vi "Delete Unicode Header.vi"(1 "String in":string) -> (0 "String out":string)   [LabVIEW 2019, in "Language Editor.lvlib"]
doc: "- - -\nCopyright (c) 2026, Merecs Engineering GmbH"
uses:
  Language Editor.lvlib
panel:
  # "Connector Pane"
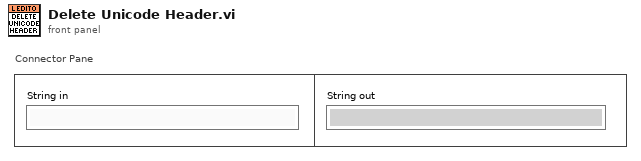
[diagram p1: front panel]
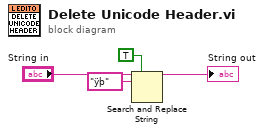
[diagram p0: block diagram]
diagram:
  n1 = Search and Replace String(replace all?=TRUE ("replace all? (F)"), input string="String in", search string="ÿþ") -> (result string=→"String out":string)  [unwired: 5 in, 3 out]
